vi "lvmcp_inodeinfo.vi"() -> ()   [LabVIEW 2015]
uses:
  <vilib>/_script/All Supported PropertiesOrMethods TypeDefs/ASPM_UniqueIDStringDatanameShortnameLongname.ctl
panel:
  out "Method":T1
  out "error out":errorcluster
  out "label":string
  out "class name":string
  in  "reference":refnum<vi>
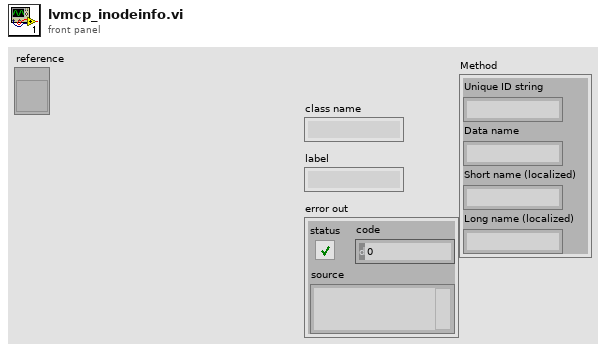
[diagram p1: front panel]
types:
  T1 = typedef "ASPM_UniqueIDStringDatanameShortnameLongname.ctl" = cluster{"Unique ID string":string, "Data name":string, "Short name (localized)":string, "Long name (localized)":string}
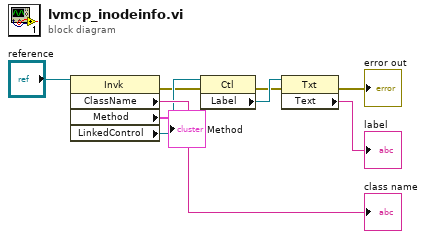
[diagram p0: block diagram]
diagram:
  n1 = property class="Invk"(reference="reference") -> (error out=w6:errorcluster, "ClassName"=→"class name":string, "Method"=→"Method":T1, "LinkedControl"=w7:refnum<vi>)  [unwired: 1 in, 1 out]
  n2 = property class="Ctl"(reference=w7, error in=w6) -> (error out=w4:errorcluster, "Label"=w5:refnum<vi>)  [unwired: 1 out]
  n3 = property class="Txt"(reference=w5, error in=w4) -> (error out=→"error out":errorcluster, "Text"=→"label":string)  [unwired: 1 out]
